vi "datasourceConfigs.to_json.vi"(8 "error in":errorcluster, 10 "datasourceConfigs":T1[](array[typedef])) -> (0 "error out":errorcluster, 2 "json":string)   [LabVIEW 2020, in "type.lvclass"]
uses:
  type.lvclass
  datasourceConfig.ctl
  7a922176-cc80-476e-b002-4975f22ae696.vi
  <vilib>/JDP Science/JSONtext/Variant to JSON Text.vi
  <vilib>/JDP Science/JSONtext/support/Format JSON Object.vi
  <vilib>/JDP Science/JSONtext/LVClass Serializer/JSONtext LVClass Serializer.lvclass
  type.lvclass/type.ctl
  <vilib>/JDP Science/JSONtext/JSONtext.lvlib
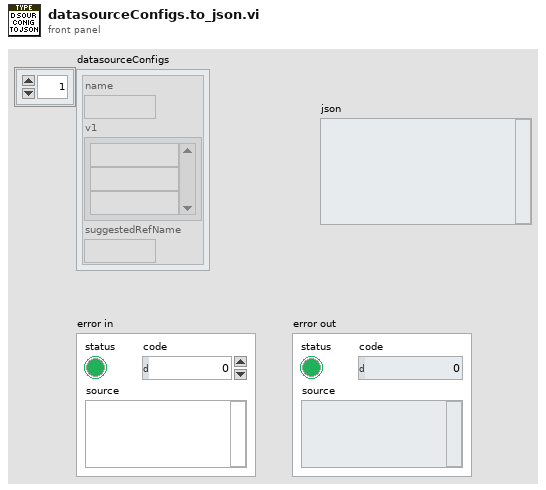
[diagram p1: front panel]
types:
  T1 = typedef "type.lvclass/datasourceConfig.ctl" = cluster{"name":string, "v1":string[], "suggestedRefName":string}
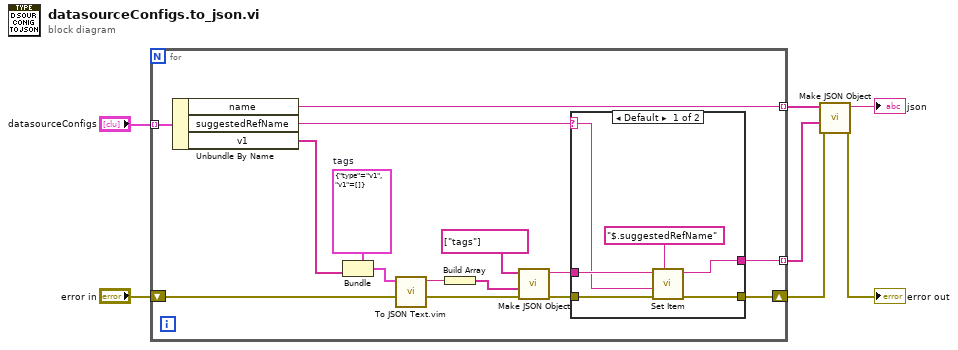
[diagram p0: block diagram]
diagram:
  n1 = for {
    tunnel: "datasourceConfigs" -> [w22] mode=indexing
    shift-right: [w14] -> w3
    shift-left: "error in" -> [w20]
    tunnel: [w15] -> w4 mode=indexing
    tunnel: [w13] -> w5 mode=indexing
    w19 = cluster{"type":string, "v1":string[]} {"type"="v1", "v1"=[]}  # tags
    n2 = Unbundle By Name(w22) -> ("name"=w13:string, "suggestedRefName"=w8:string, "v1"=w9:string[])
    n3 = Bundle(cluster=w19, "v1"=w9) -> (w21:cluster{"type":string, "v1":string[]})  [unwired: 1 in]
    n4 = call "To JSON Text.vim"("error in (no error)"=w20, "Anything"=w21) -> ("error out"=w11:errorcluster, "<JSON>"=w18:string)  [unwired: 8 in]
    n5 = Build Array(w18) -> (w17:string[])
    n6 = call <vilib>:"Make JSON Object.vi"("error in (no error)"=w11, "JSON Items"=w17, "Item Names"=string[] ["tags"]) -> ("error out"=w10:errorcluster, "<JSON>"=w12:string)  [unwired: 7 in]
    n7 = case shown="Default" w8 {
      selector: w8 -> [w23 _]
      tunnel: [w27 w30] -> w15
      tunnel: w12 -> [w28 w30]
      tunnel: w10 -> [w25 w29]
      tunnel: [w24 w29] -> w14
      frame Default {
        n8 = call <vilib>:"Set Item.vi"("$Path or Item Name"="$.suggestedRefName", "error in (no error)"=w25, "JSON to Insert"=w23, "JSON"=w28) -> ("error out"=w24:errorcluster, "<JSON>"=w27:string)  [unwired: 4 in, 1 out]
      }
      frame "" {
      }
    }
  }
  n9 = call <vilib>:"Make JSON Object.vi"("error in (no error)"=w3, "JSON Items"=w4, "Item Names"=w5) -> ("error out"=→"error out":errorcluster, "<JSON>"=→"json":string)  [unwired: 7 in]
